vi "RL.vi"(6 "error in (no error)":errorcluster, 9 "VISA session":refnum<visa-resource-name>) -> (0 "error out":errorcluster, 2 "value read":dbl format="%.7f", 3 "dup VISA session":refnum<visa-resource-name>)   [LabVIEW 2023]
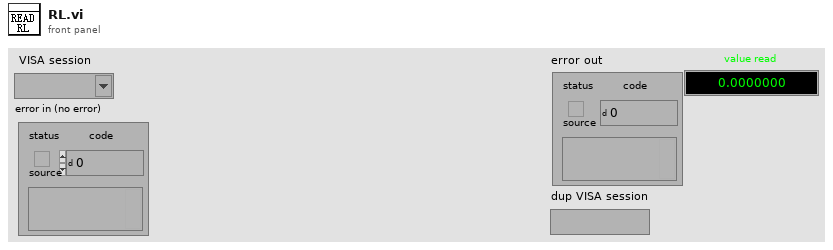
[diagram p1: front panel]
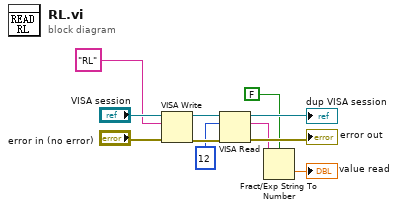
[diagram p0: block diagram]
diagram:
  n1 = VISA Write(VISA resource name="VISA session", write buffer="RL" ("输出字符串"), error in (no error)="error in (no error)") -> (VISA resource name out=w4:refnum<visa-resource-name>, error out=w9:errorcluster)  [unwired: 1 out]
  n2 = VISA Read(VISA resource name=w4, byte count=12, error in (no error)=w9) -> (VISA resource name out=→"dup VISA session":refnum<visa-resource-name>, read buffer=w6:string, error out=→"error out":errorcluster)  [unwired: 1 out]
  n3 = Fract/Exp String To Number(use system decimal point (T)=FALSE, string=w6) -> (number=→"value read":dbl)  [unwired: 2 in, 1 out]
